vi "Create GUI element.vi"(8 "error in (no error)":errorcluster, 10 "Highlight index":i32=-1, 11 "Schedule in":refnum<class "Schedule.lvclass">) -> (0 "error out":errorcluster, 2 "Array of Runs":T1 {"Number of cycles" min=1}, 3 "Schedule out":refnum<class "Schedule.lvclass">)   [LabVIEW 2020, in "Run Utilities.lvlib" / "Schedule.lvclass"]
uses:
  Schedule.lvclass
  Array of Runs - GUI.ctl
  Cell/Cell - GUI.ctl
  Run Instance/Run Instance - GUI.ctl
  Cell/Schedule Cell.lvclass
  Schedule.lvclass/Schedule.ctl
  Run Instance/Run Instance.lvclass
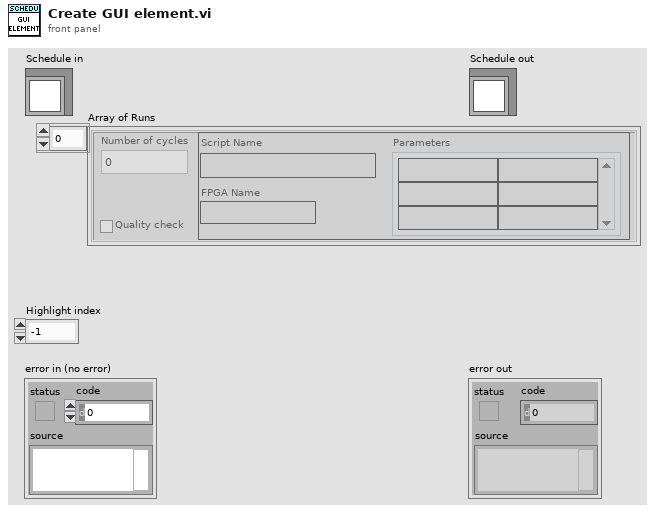
[diagram p1: front panel]
types:
  T1 = typedef "Run Utilities.lvlib/Schedule.lvclass/Array of Runs - GUI.ctl" = T2[]
  T2 = typedef "Run Utilities.lvlib/Schedule Cell.lvclass/Cell - GUI.ctl" = cluster{"Background Color":u32, "Number of cycles":u32, "Single RUN":T3, "Quality check":bool, "Cell Type":string}
  T3 = typedef "Run Utilities.lvlib/Run Instance.lvclass/Run Instance - GUI.ctl" = cluster{"Script Name":string, "Parameters":string[][], "FPGA Name":string}
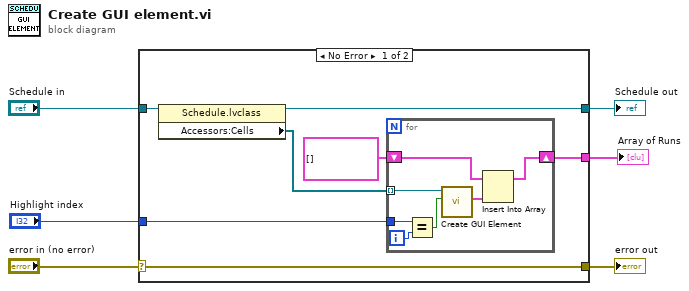
[diagram p0: block diagram]
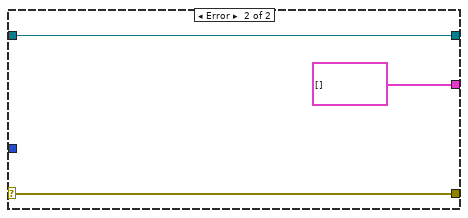
[diagram p2: hidden frame]
diagram:
  n1 = case shown="No Error" "error in (no error)" {
    selector: "error in (no error)" -> [w12 w23]
    tunnel: [w12 w23] -> w5
    tunnel: [w11 w22] -> w3
    tunnel: "Schedule in" -> [w13 w22]
    tunnel: [w8 T1 [] ("Array of Runs")] -> w2
    tunnel: "Highlight index" -> [w7 _]
    frame No Error {
      n2 = property class="Schedule.lvclass"(reference=w13) -> (reference out=w11:refnum<class "Schedule.lvclass">, "Accessors:Cells"=w9:refnum<class "Schedule Cell.lvclass">[])  [unwired: 1 in, 1 out]
      n3 = for {
        shift-right: [w19] -> w8
        shift-left: T1 [] ("Array of Runs") -> [w18]
        tunnel: w9 -> [w20] mode=indexing
        tunnel: w7 -> [w16]
        i -> [w15]
        n4 = Equal?(x=w16, y=w15) -> (x = y?=w14:bool)
        n5 = call-dynamic "Create GUI Element.vi"("Highlight"=w14, "Schedule Cell in"=w20) -> ("RUN properties"=w17:T2)  [unwired: 7 in, 2 out]
        n6 = Insert Into Array(array=w18, new element=w17) -> (w19:T1)  [unwired: 1 in]
      }
    }
    frame Error {
    }
  }
  "error out" <- w5
  "Schedule out" <- w3
  "Array of Runs" <- w2
